vi "Read Active Path.vi"(8 "error in (no error)":errorcluster, 11 "Setting Database in":refnum<class "Setting Database.lvclass">) -> (0 "error out":errorcluster, 2 "Path Settings.lvclass":refnum<class "Path Settings.lvclass">, 3 "Setting Database out":refnum<class "Setting Database.lvclass">)   [LabVIEW 2019, in "Setting Database.lvclass"]
uses:
  Setting Database.lvclass
  Path Settings/Path Settings.lvclass
  C:/Users/Albro/Documents/GitHub/AFM-Lithography/lvsrc/Classes/Settings/ObjectSettings/ObjectSettings.lvclass
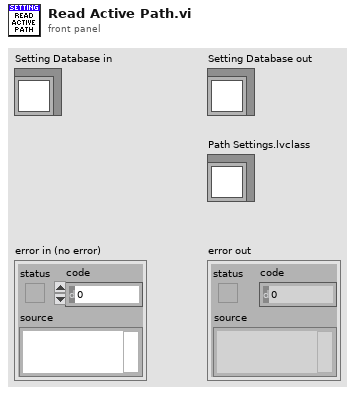
[diagram p1: front panel]
types:
  T1 = cluster{"Path":string, "Funnel":string, "Rectangle":string, "Dot":string}
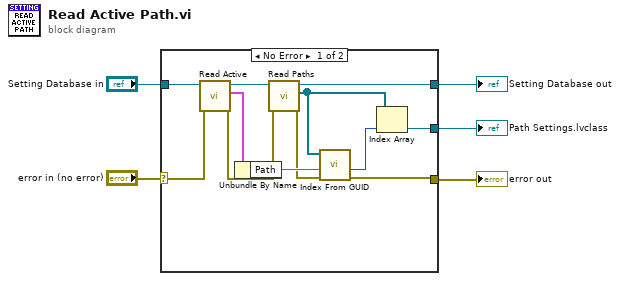
[diagram p0: block diagram]
diagram:
  n1 = case shown="No Error" "error in (no error)" {
    selector: "error in (no error)" -> [w12 w18]
    tunnel: [w6 w18] -> w4
    tunnel: [w16 w19] -> w2
    tunnel: "Setting Database in" -> [w14 w19]
    tunnel: [w17 _] -> w1
    frame No Error {
      n2 = call "Read Active.vi"("error in (no error)"=w12, "Setting Database in"=w14) -> ("error out"=w11:errorcluster, "Active"=w13:T1, "Setting Database out"=w15:refnum<class "Setting Database.lvclass">)  [unwired: 7 in]
      n3 = Unbundle By Name(w13) -> ("Path"=w10:string)
      n4 = call "Read Paths.vi"("error in (no error)"=w11, "Setting Database in"=w15) -> ("error out"=w7:errorcluster, "Paths"=w8:refnum<class "Path Settings.lvclass">[], "Setting Database out"=w16:refnum<class "Setting Database.lvclass">)  [unwired: 7 in]
      n5 = call "Index From GUID.vi"("error in"=w7, "GUID"=w10, "Objects In"=w8) -> ("error out"=w6:errorcluster, "Index"=w9:i32)  [unwired: 5 in, 2 out]
      n6 = Index Array(array=w8, index=w9) -> (element=w17:refnum<class "Path Settings.lvclass">)
    }
    frame Error {
    }
  }
  "error out" <- w4
  "Setting Database out" <- w2
  "Path Settings.lvclass" <- w1
